vi "Get Section Names.vi"(8 "error in (no error)":errorcluster, 11 "Config in":T1) -> (0 "error out":errorcluster, 1 "Section Names":string[](array[string]), 3 "Config out":T1)   [LabVIEW 2017, in "LabVIEW-Config.lvlib"]
uses:
  LabVIEW-Config.lvlib
  Config.ctl
  LineToken.ctl
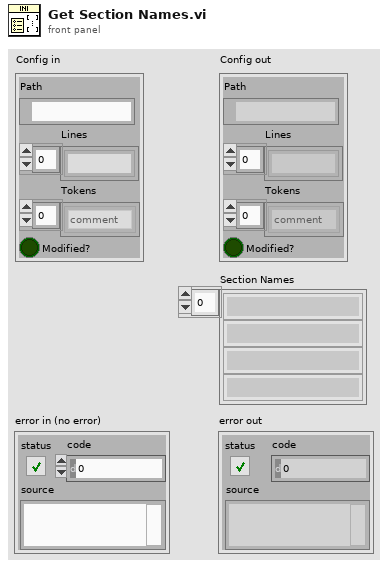
[diagram p1: front panel]
types:
  T1 = typedef "LabVIEW-Config.lvlib/Config.ctl" = cluster{"Path":path, "Lines":string[], "Tokens":T2[], "Modified?":bool}
  T2 = typedef "LabVIEW-Config.lvlib/LineToken.ctl" = enum8{"comment", "section", "key", "more"}
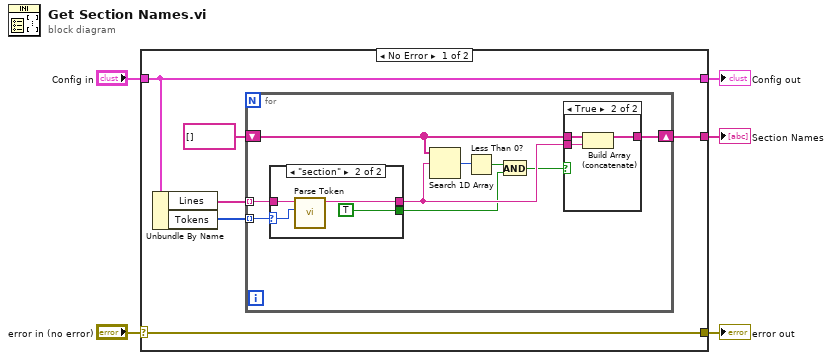
[diagram p0: block diagram]
diagram:
  n1 = case shown="No Error" "error in (no error)" {
    selector: "error in (no error)" -> [w9 w30]
    tunnel: "Config in" -> [w8 w29]
    tunnel: [w6 _] -> w4
    tunnel: [w9 w30] -> w3
    tunnel: [w8 w29] -> w1
    frame No Error {
      n2 = Unbundle By Name(w8) -> ("Lines"=w10:string[], "Tokens"=w11:T2[])
      n3 = for {
        tunnel: w11 -> [w20] mode=indexing
        tunnel: w10 -> [w19] mode=indexing
        shift-right: [w18] -> w6
        shift-left: string[] [] -> [w17]
        n4 = case shown="\"section\"" w20 {
          selector: w20 -> [_ w26]
          tunnel: w19 -> [_ w27]
          tunnel: [_ w25] -> w16
          tunnel: [_ TRUE] -> w13
          frame Default {
          }
          frame "section" {
            n5 = call "Parse Token.vi"("Token"=w26, "Line"=w27) -> ("Name"=w25:string)  [unwired: 8 in, 1 out]
          }
        }
        n6 = Search 1D Array(1D array=w17, element=w16) -> (index of element=w15:i32)  [unwired: 1 in]
        n7 = Less Than 0?(x=w15) -> (x < 0?=w14:bool)
        n8 = And(x=w14, y=w13) -> (x .and. y?=w12:bool)
        n9 = case shown="True" w12 {
          tunnel: [w21 w24] -> w18
          tunnel: w17 -> [w21 w23]
          tunnel: w16 -> [_ w22]
          frame False {
          }
          frame True {
            n10 = Build Array (concatenate)(w23, w22) -> (w24:string[])
          }
        }
      }
    }
    frame Error {
    }
  }
  "error out" <- w3
  "Config out" <- w1
  "Section Names" <- w4
